vi "Layout Subpanels.vi"(8 "error in (no error)":errorcluster, 10 "Panels in":refnum<class "ArrayPanel.lvclass">[][](array[class]), 11 "2DArrayManager in":refnum<class "2DArrayManager.lvclass">) -> (0 "error out":errorcluster, 2 "Used SubPanels":refnum<vi>[](array[refnum]), 3 "2DArrayManager out":refnum<class "2DArrayManager.lvclass">, 5 "Insufficient Subpanels":bool)   [LabVIEW 2020, in "OOPanel.lvlib" / "2DArrayManager.lvclass"]
uses:
  2DArrayManager.lvclass
  ArrayPanel/ArrayPanel.lvclass
  C:/dev/lv20CE/relink/lv-oopanel/OOPanel/Panel/Panel.lvclass
  2DArrayManager.lvclass/2DArrayManager.ctl
  2DPanelBlank/State.ctl
  2DPanelBlank/2DPanelBlank.lvclass/2DPanelBlank.ctl
  2DPanelBlank/2DPanelBlank.lvclass
  Manager/Manager.lvclass
  Panel/Panel.lvclass
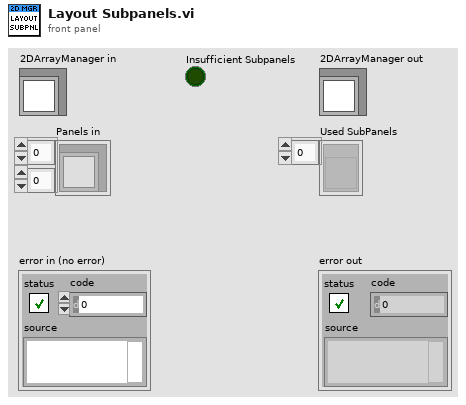
[diagram p1: front panel]
types:
  T1 = typedef "OOPanel.lvlib/2DPanelBlank.lvclass/State.ctl" = enum16{"New", "Idle", "Pool", "Used", "No SP"}
  T2 = typedef "OOPanel.lvlib/Visibility State.ctl" = enum16{"Idle", "Closed", "Hidden", "Visible", "Subpanel", "Hidden Subpanel"}
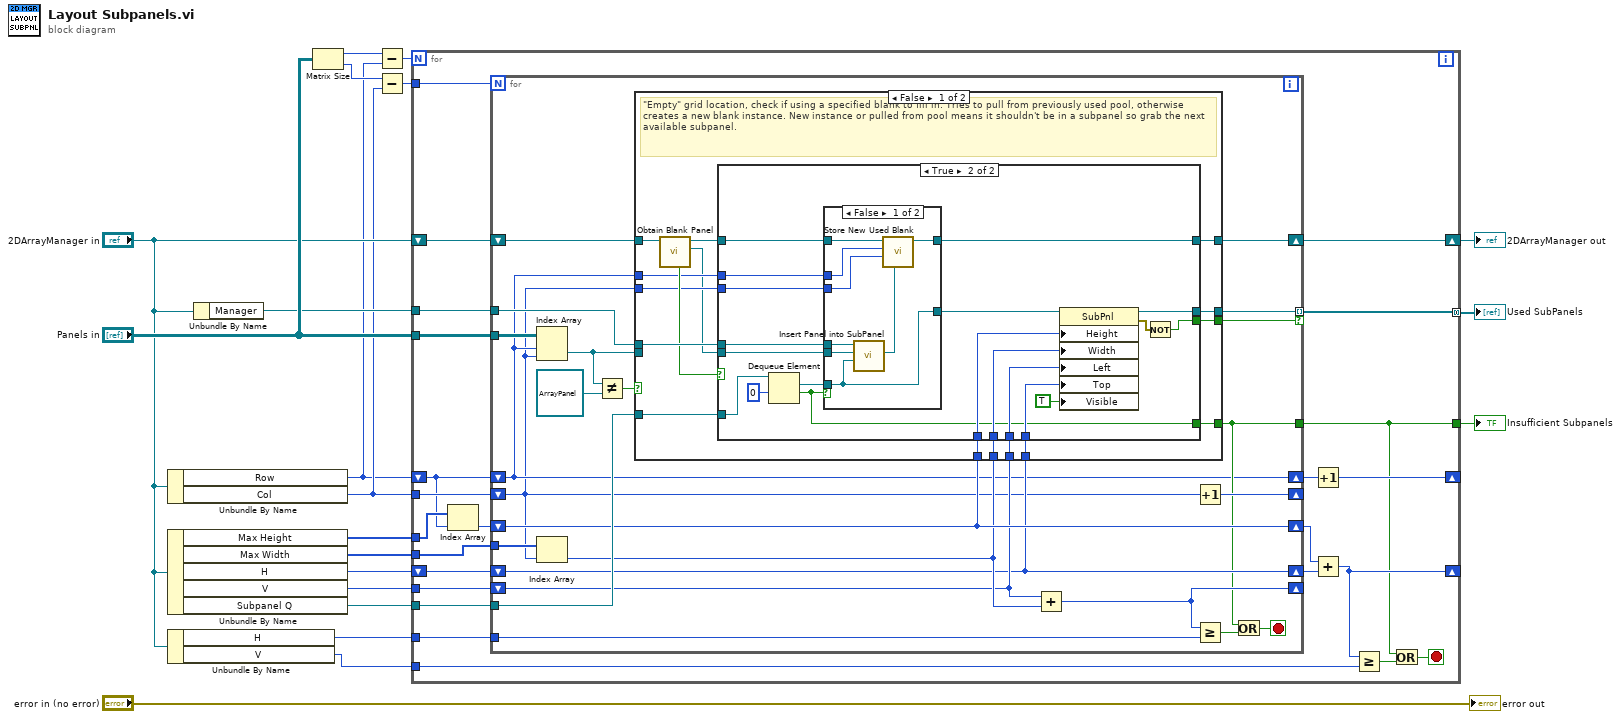
[diagram p0: block diagram]
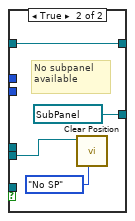
[diagram p3: hidden frame]
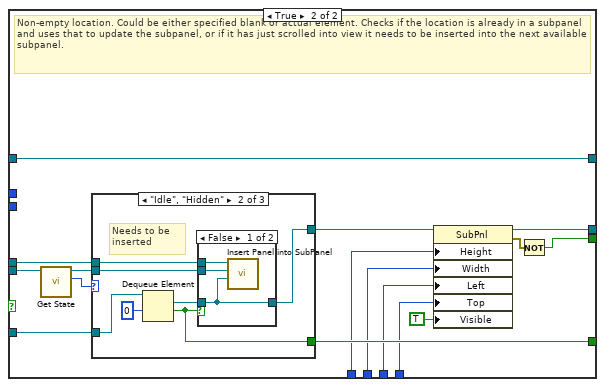
[diagram p4: hidden frame]
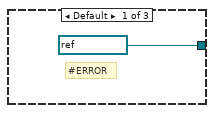
[diagram p5: hidden frame]
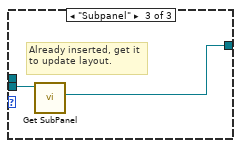
[diagram p7: hidden frame]
diagram:
  n1 = Unbundle By Name("2DArrayManager in") -> ("Row"=w1:i32, "Col"=w2:i32)
  n2 = Unbundle By Name("2DArrayManager in") -> ("Max Height"=w12:i32[], "Max Width"=w11:i32[], "H"=w14:i32, "V"=w13:i32, "Subpanel Q"=w8:refnum<queue>)
  n3 = Unbundle By Name("2DArrayManager in") -> ("H"=w10:i32, "V"=w9:i32)
  n4 = Unbundle By Name("2DArrayManager in") -> ("Manager"=w3:refnum<class "Manager.lvclass">)
  n5 = Matrix Size(0:"Panels in") -> (1:w19:i32, 2:w17:i32)
  n6 = Subtract(x=w19, y=w1) -> (x-y=w18:i32)
  n7 = Subtract(x=w17, y=w2) -> (x-y=w16:i32)
  n8 = for {
    N: w18 -> [_]
    tunnel: w16 -> [w44]
    tunnel: "Panels in" -> [w43]
    shift-right: [w40] -> _
    shift-left: w1 -> [w34]
    tunnel: w2 -> [w39]
    shift-right: [w30] -> _
    shift-left: w14 -> [w38]
    tunnel: w12 -> [w35]
    tunnel: w11 -> [w36]
    tunnel: w13 -> [w37]
    tunnel: w10 -> [w31]
    tunnel: w9 -> [w29]
    tunnel: w8 -> [w42]
    tunnel: [w26] -> w7
    tunnel: [w25] -> w6 mode=concatenating
    shift-right: [w23] -> w5
    shift-left: "2DArrayManager in" -> [w24]
    tunnel: w3 -> [w22]
    stop <- w27 stop-if-true
    n9 = Index Array(array=w35, index=w34) -> (element=w33:i32)
    n10 = for {
      N: w44 -> [_]
      tunnel: w43 -> [w67]
      shift-right: [w46] -> w41
      shift-left: w34 -> [w46]
      shift-right: [w65] -> _
      shift-left: w39 -> [w45]
      shift-right: [w55] -> w32
      shift-left: w38 -> [w55]
      shift-right: [w54] -> _
      shift-left: w37 -> [w56]
      tunnel: w36 -> [w64]
      shift-right: [w58] -> w21
      shift-left: w33 -> [w58]
      tunnel: w31 -> [w63]
      tunnel: w42 -> [w66]
      tunnel: [w53] -> w26
      tunnel: [w52] -> w25 mode=indexing if=w51
      shift-right: [w49] -> w23
      shift-left: w24 -> [w50]
      tunnel: w22 -> [w48]
      stop <- w61 stop-if-true
      n11 = Index Array(array=w67, index (row)=w46, index (col)=w45) -> (element=w47:refnum<class "ArrayPanel.lvclass">)
      n12 = Index Array(array=w64, index=w45) -> (element=w57:i32)
      n13 = Not Equal?(x=w47, y=refnum<class "ArrayPanel.lvclass"> refnum) -> (x != y?=w59:bool)
      n14 = case shown="False" w59 {
        tunnel: w48 -> [w82 w131]
        tunnel: w47 -> [_ w117]
        tunnel: w66 -> [w70 w130]
        tunnel: w58 -> [w76 w125]
        tunnel: w57 -> [w77 w124]
        tunnel: w56 -> [w78 w123]
        tunnel: w55 -> [w79 w122]
        tunnel: [w69 w129] -> w53
        tunnel: [w81 w118] -> w52
        tunnel: [w80 w120] -> w51
        tunnel: w50 -> [w83 w119]
        tunnel: [w74 w119] -> w49
        tunnel: w46 -> [w72 _]
        tunnel: w45 -> [w71 _]
        frame False {
          # "\"Empty\" grid location, check if using a specified blank to fill in. Tries to pull from previously used pool, otherwise creates a new blank instance. New instance or pulled from pool means it shouldn't be in a subpanel so grab the next available subpanel."
          n15 = call "Obtain Blank Panel.vi"("2DArrayManager in"=w83) -> ("Blank"=w68:refnum<class "2DPanelBlank.lvclass">, "2DArrayManager out"=w75:refnum<class "2DArrayManager.lvclass">, "Use Blank"=w73:bool)  [unwired: 7 in, 1 out]
          n16 = case shown="True" w73 {
            tunnel: w82 -> [_ w103]
            tunnel: w68 -> [_ w102]
            tunnel: [_ w99] -> w81
            tunnel: [_ w98] -> w80
            tunnel: w79 -> [_ w97]
            tunnel: w78 -> [_ w96]
            tunnel: w77 -> [_ w95]
            tunnel: w76 -> [_ w94]
            tunnel: w75 -> [w84 w89]
            tunnel: [w84 w88] -> w74
            tunnel: w72 -> [_ w87]
            tunnel: w71 -> [_ w86]
            tunnel: w70 -> [_ w92]
            tunnel: [_ w85] -> w69
            frame False {
            }
            frame True {
              n17 = Dequeue Element(queue=w92, timeout in ms (-1)=0) -> (element=w91:refnum<vi>, timed out?=w85:bool)  [unwired: 1 in, 2 out]
              n18 = case shown="False" w85 {
                tunnel: w103 -> [w111 _]
                tunnel: w102 -> [w110 w113]
                tunnel: w91 -> [w109 _]
                tunnel: [w109 refnum<vi> refnum ("target class")] -> w90
                tunnel: w89 -> [w108 w114]
                tunnel: [w107 w114] -> w88
                tunnel: w87 -> [w105 _]
                tunnel: w86 -> [w104 _]
                frame False {
                  n19 = call "Insert Panel into SubPanel.vi"("SubPanel"=w109, "Panel In"=w110, "Manager in"=w111) -> ("Panel"=w106:refnum<class "2DPanelBlank.lvclass">)  [unwired: 6 in, 2 out]
                  n20 = call "Store New Used Blank.vi"("2DPanelBlank"=w106, "Col"=w104, "Row"=w105, "2DArrayManager in"=w108) -> ("2DArrayManager out"=w107:refnum<class "2DArrayManager.lvclass">)  [unwired: 6 in, 1 out]
                }
                frame True {
                  # "No subpanel available"
                  n21 = call "Clear Position.vi"("State"=State."No SP", "2DPanelBlank in"=w113) -> ()  [unwired: 8 in, 2 out]
                }
              }
              n22 = property class="SubPnl"(reference=w90, "Height"=w94, "Width"=w95, "Left"=w96, "Top"=w97, "Visible"=TRUE) -> (reference out=w99:refnum<vi>, error out=w100:errorcluster)  [unwired: 1 in]
              n23 = Not(x=w100) -> (.not. x?=w98:bool)
            }
          }
        }
        frame True {
          # "Non-empty location. Could be either specified blank or actual element. Checks if the location is already in a subpanel and uses that to update the subpanel, or if it has just scrolled into view it needs to be inserted into the next available subpanel."
          n24 = call "Get State.vi"("Panel in"=w117) -> ("State"=w127:T2, "Panel out"=w128:refnum<class "ArrayPanel.lvclass">)  [unwired: 8 in, 1 out]
          n25 = case shown="\"Idle\", \"Hidden\"" w127 {
            tunnel: w131 -> [_ w139 _]
            tunnel: w130 -> [_ w138 _]
            tunnel: [_ w135 _] -> w129
            tunnel: w128 -> [_ w134 w144]
            tunnel: [refnum<vi> refnum ("SubPanel") w133 w143] -> w116
            frame Default {
              # "#ERROR"
            }
            frame "Idle", "Hidden" {
              # "Needs to be inserted"
              n26 = Dequeue Element(queue=w138, timeout in ms (-1)=0) -> (element=w136:refnum<vi>, timed out?=w135:bool)  [unwired: 1 in, 2 out]
              n27 = case shown="False" w135 {
                tunnel: w139 -> [w142 _]
                tunnel: w134 -> [w141 _]
                tunnel: w136 -> [w140 _]
                tunnel: [w140 _] -> w133
                frame False {
                  n28 = call "Insert Panel into SubPanel.vi"("SubPanel"=w140, "Panel In"=w141, "Manager in"=w142) -> ()  [unwired: 6 in, 3 out]
                }
                frame True {
                }
              }
            }
            frame "Subpanel" {
              # "Already inserted, get it to update layout."
              n29 = call "Get SubPanel.vi"("Panel in"=w144) -> ("SubPanel"=w143:refnum<vi>)  [unwired: 8 in, 2 out]
            }
          }
          n30 = property class="SubPnl"(reference=w116, "Height"=w125, "Width"=w124, "Left"=w123, "Top"=w122, "Visible"=TRUE) -> (reference out=w118:refnum<vi>, error out=w121:errorcluster)  [unwired: 1 in]
          n31 = Not(x=w121) -> (.not. x?=w120:bool)
        }
      }
      n32 = Add(x=w56, y=w57) -> (x+y=w54:i32)
      n33 = Increment(x=w45) -> (x+1=w65:i32)
      n34 = Greater Or Equal?(x=w54, y=w63) -> (x >= y?=w62:bool)
      n35 = Or(x=w53, y=w62) -> (x .or. y?=w61:bool)
    }
    n36 = Increment(x=w41) -> (x+1=w40:i32)
    n37 = Add(x=w21, y=w32) -> (x+y=w30:i32)
    n38 = Greater Or Equal?(x=w30, y=w29) -> (x >= y?=w28:bool)
    n39 = Or(x=w26, y=w28) -> (x .or. y?=w27:bool)
  }
  "2DArrayManager out" <- w5
  "Insufficient Subpanels" <- w7
  "Used SubPanels" <- w6
  "error out" <- "error in (no error)"
